vi "FuncVI-_STDev.vi"(5 "InstanceRef":T2, 9 "arg list":T1[](array[typedef]) {"num" format="%.2f"}) -> (0 "error out":bool, 3 "result":T1 {"num" format="%.2f"})   [LabVIEW 2021]
doc: "::: CalcExpress Toolkit :::\nCopyright (c) 2000-2026 Konstantin Shifershteyn. All rights reserved."
uses:
  cetypes.llb/CalcExpress Function Argument Info.ctl
  cetypes.llb/CalcExpress Instance RefNum.ctl
  <vilib>/Analysis/NI_AALBase.lvlib
panel:
  in  "max arg num":i32=1
  in  "min arg num":i32=1
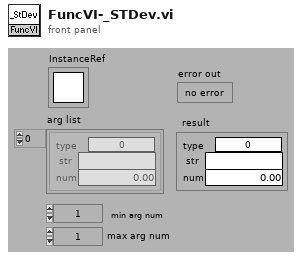
[diagram p1: front panel]
types:
  T1 = typedef "CalcExpress Function Argument Info.ctl" = cluster{"type":u32, "str":string, "num":dbl}
  T2 = typedef "CalcExpress Instance RefNum.ctl" = refnum<k1>
  T3 = enum32{"String", "DBL Number", "identifier", "1D Array of DBL", "2D Array of DBL", "CDB Number", "1D Array of CDB", "2D Array of CDB", "1D Array of String", "2D Array of String", "Unknown data type"}
  T4 = cluster{"use this constant to specify a predefined type":enum32{"String", "DBL Number", "identifier", "1D Array of DBL", "2D Array of DBL", "CDB Number", "1D Array of CDB", "2D Array of CDB", "1D Array of String", "2D Array of String", "Unknown data type"}, string, "standard deviation":dbl}
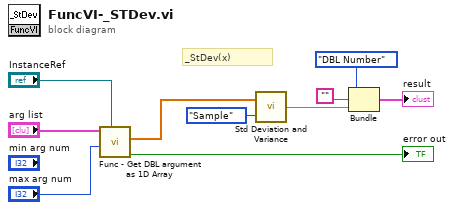
[diagram p0: block diagram]
diagram:
  # "_StDev(x)"
  n1 = call "Func - Get DBL argument as 1D Array.vi"("InstanceRef"="InstanceRef", "max arg num"="max arg num", "arg list"="arg list") -> ("error out"=→"error out":bool, "1D data"=w10:dbl[])  [unwired: 5 in, 2 out]
  n2 = call <vilib>:"Std Deviation and Variance.vi"("X"=w10, "Weighting (Sample)"=enum16{"Sample", "Population"}."Sample") -> ("standard deviation"=w7:dbl)  [unwired: 2 out]
  n3 = Bundle("use this constant to specify a predefined type"=T3."DBL Number", "", "standard deviation"=w7) -> (→"result":T4)  [unwired: 1 in]
